vi "WriteRegAck.vi"(6 "error in":errorcluster, 7 "value in":i32, 8 "string in":string, 9 "connection ID in":refnum<k5>) -> (0 "error out":errorcluster, 1 "number out":i32, 2 "Error":bool=TRUE, 3 "connection ID out":refnum<k5>, 5 "string out":string)   [LabVIEW 2020]
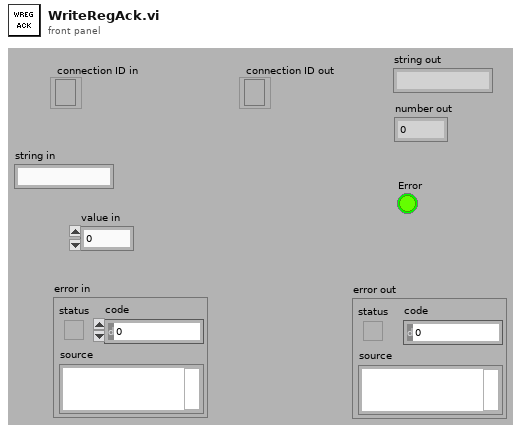
[diagram p1: front panel]
types:
  T1 = enum16{"Standard", "Buffered", "CRLF", "Immediate"}
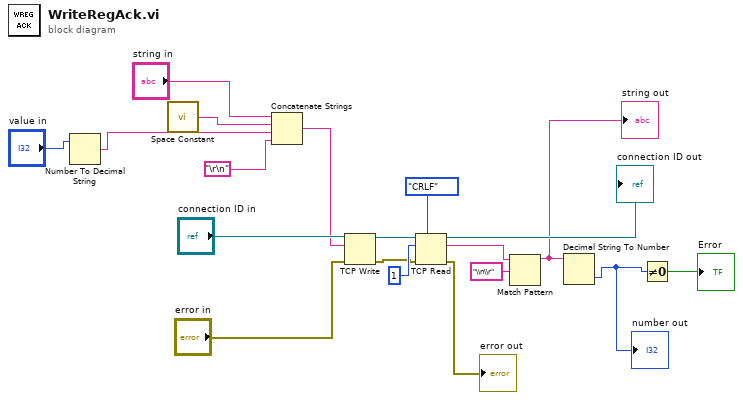
[diagram p0: block diagram]
diagram:
  n1 = Number To Decimal String(number="value in") -> (decimal integer string=w7:string)  [unwired: 1 in]
  n2 = call <vilib>:"Space Constant.vi"() -> ("String"=w5:string)
  n3 = Concatenate Strings("string in", w5, w7, "\r\n") -> (w4:string)
  n4 = TCP Write(connection ID="connection ID in", data in=w4, error in (no error)="error in") -> (connection ID out=w19:refnum<k5>, error out=w11:errorcluster)  [unwired: 1 in, 1 out]
  n5 = TCP Read(connection ID=w19, bytes to read=1, error in (no error)=w11, 7:T1."CRLF" ("mode (standard)")) -> (connection ID out=→"connection ID out":refnum<k5>, data out=w15:string, error out=→"error out":errorcluster)  [unwired: 1 in]
  n6 = Match Pattern(string=w15, regular expression="\\n\\r") -> (before substring=w1:string)  [unwired: 1 in, 3 out]
  "string out" <- w1
  n7 = Decimal String To Number(string=w1) -> (number=w2:i32)  [unwired: 2 in, 1 out]
  "number out" <- w2
  n8 = Not Equal To 0?(x=w2) -> (x != 0?=→"Error":bool)
